vi "Prefilter.60Hz_Notch.vi"(8 "error in (no error)":errorcluster, 10 "signal in":waveform(dbl)[](array[waveform]), 11 "DSP in":refnum<class "DSP.lvclass">) -> (0 "error out":errorcluster, 2 "signal out":waveform(dbl)[](array[waveform]), 3 "DSP out":refnum<class "DSP.lvclass">)   [LabVIEW 2019, in "DSP.lvclass"]
uses:
  DSP.lvclass
  DSP.lvclass/DSP.ctl
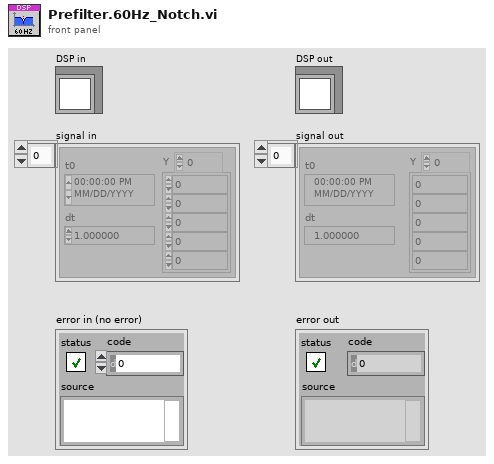
[diagram p1: front panel]
types:
  T1 = cluster{"filter structure":enum32{"IIR 2nd Order", "IIR 4th Order"}, "Reverse Coefficients":dbl[], "Forward Coefficients":dbl[]}[]
  T2 = cluster{"filter structure":enum32{"IIR 2nd Order", "IIR 4th Order"}, "Reverse Coefficients":dbl[], "Forward Coefficients":dbl[]}
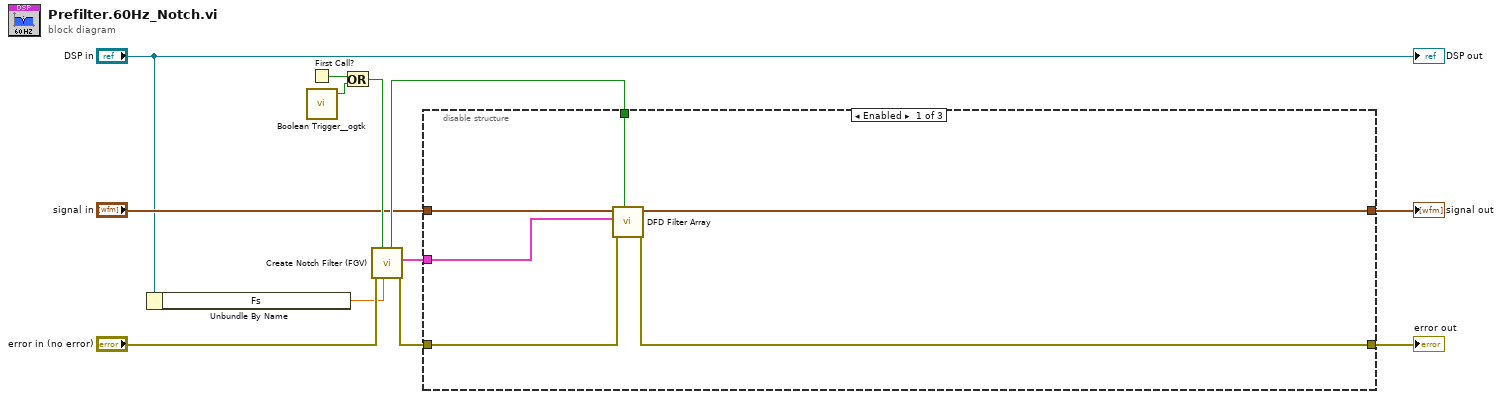
[diagram p0: block diagram]
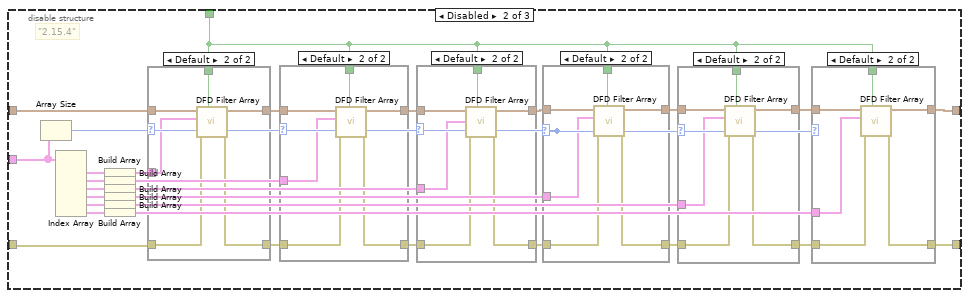
[diagram p2: hidden frame]
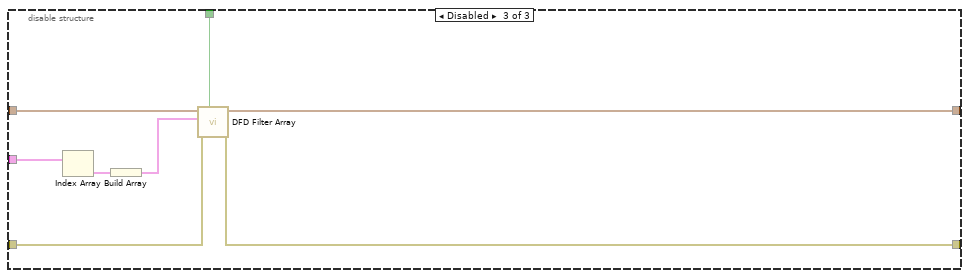
[diagram p9: hidden frame]
diagram:
  n1 = Unbundle By Name("DSP in") -> ("Fs"=w1:dbl)
  n2 = First Call?() -> (First Call?: T/F=w10:bool)
  n3 = call <userlib>:"Boolean Trigger__ogtk.vi"() -> ("Rising Edge"=w8:bool)  [unwired: 2 in, 1 out]
  n4 = Or(x=w10, y=w8) -> (x .or. y?=w9:bool)
  n5 = call "Create Notch Filter (FGV).vi"("fs (Hz)"=w1, "init [F]"=w9, "error in (no error)"="error in (no error)") -> ("error out"=w5:errorcluster, "IIR Filters"=w7:T1, "init?"=w6:bool)  [unwired: 6 in]
  n6 = disable-structure shown="Enabled" {
    disable-tunnel: [w18 w35 w102] -> w3
    disable-tunnel: [w17 w37 w99] -> w11
    disable-tunnel: w5 -> [w16 w32 w100]
    disable-tunnel: "signal in" -> [w15 w36 w103]
    disable-tunnel: w7 -> [w13 w31 w98]
    disable-tunnel: w6 -> [w14 w34 w101]
    frame Enabled {
      n7 = call "DFD Filter Array.vi"("init (F)"=w14, "error in (no error)"=w16, "IIR Filters"=w13, "signal in"=w15) -> ("error out"=w17:errorcluster, "signal out"=w18:waveform(dbl)[])  [unwired: 6 in]
    }
    frame Disabled {
      # "\"2.15.4\""
      n8 = Array Size(array=w31) -> (size(s)=w33:i32)
      n9 = Index Array(array=w31) -> (element #1=w30:T2, element #2=w28:T2, element #3=w27:T2, element #4=w19:T2, element #5=w20:T2, element #6=w26:T2)  [unwired: 6 in]
      n10 = Build Array(w30) -> (w29:T1)
      n11 = Build Array(w28) -> (w25:T1)
      n12 = Build Array(w27) -> (w24:T1)
      n13 = Build Array(w19) -> (w23:T1)
      n14 = Build Array(w20) -> (w22:T1)
      n15 = Build Array(w26) -> (w21:T1)
      n16 = case shown="Default" w33 {
        tunnel: [w49 w55] -> w44
        tunnel: [w48 w54] -> w45
        tunnel: w36 -> [w49 w53]
        tunnel: w34 -> [_ w52]
        tunnel: w32 -> [w48 w51]
        tunnel: w29 -> [_ w50]
        frame 0 {
        }
        frame Default {
          n17 = call "DFD Filter Array.vi"("init (F)"=w52, "error in (no error)"=w51, "IIR Filters"=w50, "signal in"=w53) -> ("error out"=w54:errorcluster, "signal out"=w55:waveform(dbl)[])  [unwired: 6 in]
        }
      }
      n18 = case shown="Default" w33 {
        tunnel: [w57 w63] -> w38
        tunnel: [w56 w62] -> w43
        tunnel: w44 -> [w57 w61]
        tunnel: w45 -> [w56 w60]
        tunnel: w34 -> [_ w59]
        tunnel: w25 -> [_ w58]
        frame 0, 1 {
        }
        frame Default {
          n19 = call "DFD Filter Array.vi"("init (F)"=w59, "error in (no error)"=w60, "IIR Filters"=w58, "signal in"=w61) -> ("error out"=w62:errorcluster, "signal out"=w63:waveform(dbl)[])  [unwired: 6 in]
        }
      }
      n20 = case shown="Default" w33 {
        tunnel: w38 -> [w64 w71]
        tunnel: [w64 w70] -> w39
        tunnel: [w65 w69] -> w41
        tunnel: w43 -> [w65 w68]
        tunnel: w34 -> [_ w67]
        tunnel: w24 -> [_ w66]
        frame 0..2 {
        }
        frame Default {
          n21 = call "DFD Filter Array.vi"("init (F)"=w67, "error in (no error)"=w68, "IIR Filters"=w66, "signal in"=w71) -> ("error out"=w69:errorcluster, "signal out"=w70:waveform(dbl)[])  [unwired: 6 in]
        }
      }
      n22 = case shown="Default" w33 {
        tunnel: w39 -> [w73 w79]
        tunnel: [w73 w78] -> w40
        tunnel: w41 -> [w72 w76]
        tunnel: [w72 w77] -> w42
        tunnel: w34 -> [_ w75]
        tunnel: w23 -> [_ w74]
        frame 0..3 {
        }
        frame Default {
          n23 = call "DFD Filter Array.vi"("init (F)"=w75, "error in (no error)"=w76, "IIR Filters"=w74, "signal in"=w79) -> ("error out"=w77:errorcluster, "signal out"=w78:waveform(dbl)[])  [unwired: 6 in]
        }
      }
      n24 = case shown="Default" w33 {
        tunnel: [w80 w87] -> w47
        tunnel: w40 -> [w81 w86]
        tunnel: w42 -> [w80 w84]
        tunnel: [w81 w85] -> w46
        tunnel: w34 -> [_ w83]
        tunnel: w22 -> [_ w82]
        frame 0..4 {
        }
        frame Default {
          n25 = call "DFD Filter Array.vi"("init (F)"=w83, "error in (no error)"=w84, "IIR Filters"=w82, "signal in"=w86) -> ("error out"=w87:errorcluster, "signal out"=w85:waveform(dbl)[])  [unwired: 6 in]
        }
      }
      n26 = case shown="Default" w33 {
        tunnel: [w88 w95] -> w37
        tunnel: w46 -> [w89 w94]
        tunnel: w47 -> [w88 w92]
        tunnel: [w89 w93] -> w35
        tunnel: w34 -> [_ w91]
        tunnel: w21 -> [_ w90]
        frame 0..5 {
        }
        frame Default {
          n27 = call "DFD Filter Array.vi"("init (F)"=w91, "error in (no error)"=w92, "IIR Filters"=w90, "signal in"=w94) -> ("error out"=w95:errorcluster, "signal out"=w93:waveform(dbl)[])  [unwired: 6 in]
        }
      }
    }
    frame Disabled {
      n28 = Index Array(array=w98) -> (element=w97:T2)  [unwired: 1 in]
      n29 = Build Array(w97) -> (w96:T1)
      n30 = call "DFD Filter Array.vi"("init (F)"=w101, "error in (no error)"=w100, "IIR Filters"=w96, "signal in"=w103) -> ("error out"=w99:errorcluster, "signal out"=w102:waveform(dbl)[])  [unwired: 6 in]
    }
  }
  "error out" <- w11
  "signal out" <- w3
  "DSP out" <- "DSP in"
